vi "Create Groups.vi"(7 "Group":bool, 8 "error in (no error)":errorcluster, 11 "Channels":T1[](array[typedef]) {"Data Type" format="%.0x"}) -> (0 "error out":errorcluster, 3 "Channels out":T1[](array[typedef]) {"Data Type" format="%.0x"})   [LabVIEW 2020, in "FPGA Addon System Explorer.lvlib"]
uses:
  FPGA Addon System Explorer.lvlib
  Addon Shared/Types/Register Information.ctl
  Addon Shared/Types/FPGA Addon Data Type.ctl
  Addon Shared/FPGA Addon Shared.lvlib
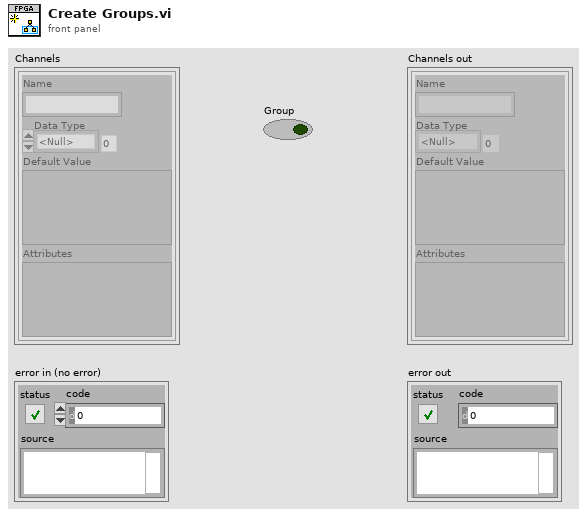
[diagram p1: front panel]
types:
  T1 = typedef "FPGA Addon Shared.lvlib/Register Information.ctl" = cluster{"Name":string, "Data Type":T2, "Default Value":variant, "Attributes":variant}
  T2 = typedef "FPGA Addon Shared.lvlib/FPGA Addon Data Type.ctl" = enum8{"<Null>", "I8", "I16", "I32", "I64", "U8", "U16", "U32", "U64", "SGL", "Boolean", "Analog PWM In Settings", "Analog PWM In", "Digital PWM In Settings", "Digital PWM In", "Digital PWM Out", "Sine Out", "FXP", "FXP+/-24.5", "FXP+/-16.5", "FXP+/-32.8", "FXP+/-64.32", "FXP+/-16.7", "FXP+/-20.5", "FXP+/-27.5", "FXP+/-32.16", "FXP+16.3", "FXP+18.3", "Digital Static In", "Digital Static Out", "Digital Static In Settings", "Digital WSS Out", "Quad Encoder Settings", "Quad Encoder In", "Group"}
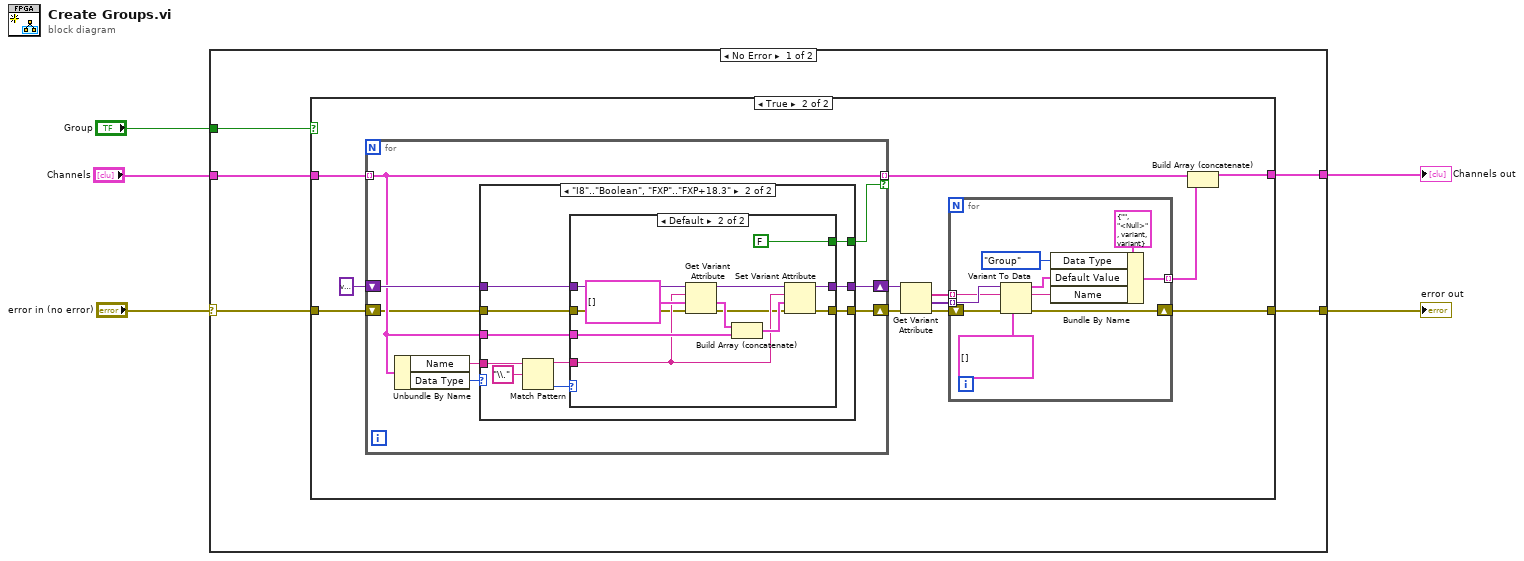
[diagram p0: block diagram]
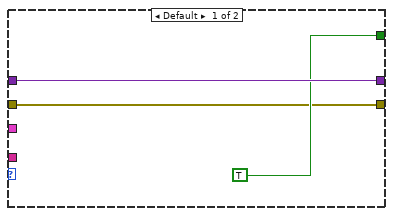
[diagram p3: hidden frame]
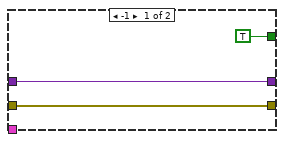
[diagram p4: hidden frame]
diagram:
  n1 = case shown="No Error" "error in (no error)" {
    selector: "error in (no error)" -> [w6 w70]
    tunnel: [w10 w71] -> w5
    tunnel: "Channels" -> [w9 w71]
    tunnel: [w8 w70] -> w3
    tunnel: "Group" -> [w7 _]
    frame No Error {
      n2 = case shown="True" w7 {
        tunnel: w9 -> [w11 w24]
        tunnel: w6 -> [w12 w17]
        tunnel: [w12 w16] -> w8
        tunnel: [w11 w15] -> w10
        frame False {
        }
        frame True {
          n3 = for {
            tunnel: w24 -> [w37] mode=indexing
            shift-right: [w38] -> w22
            shift-left: variant -> [w39]
            tunnel: [w37] -> w14 mode=indexing if=w36
            shift-right: [w35] -> w19
            shift-left: w17 -> [w34]
            n4 = Unbundle By Name(w37) -> ("Name"=w41:string, "Data Type"=w40:T2)
            n5 = case shown="\"I8\"..\"Boolean\", \"FXP\"..\"FXP+18.3\"" w40 {
              tunnel: w41 -> [_ w54]
              tunnel: w39 -> [w44 w51]
              tunnel: w37 -> [_ w49]
              tunnel: [w44 w48] -> w38
              tunnel: [TRUE w47] -> w36
              tunnel: [w42 w46] -> w35
              tunnel: w34 -> [w42 w45]
              frame Default {
              }
              frame "I8".."Boolean", "FXP".."FXP+18.3" {
                n6 = Match Pattern(string=w54, regular expression="\\.") -> (before substring=w50:string, offset past match=w52:i32)  [unwired: 1 in, 2 out]
                n7 = case shown="Default" w52 {
                  tunnel: w51 -> [w57 w69]
                  tunnel: w50 -> [_ w64]
                  tunnel: w49 -> [_ w66]
                  tunnel: [w57 w63] -> w48
                  tunnel: [TRUE FALSE] -> w47
                  tunnel: [w55 w61] -> w46
                  tunnel: w45 -> [w55 w60]
                  frame -1 {
                  }
                  frame Default {
                    n8 = Get Variant Attribute(Variant=w69, name=w64, default value (empty Variant)=T1[] [], error in=w60) -> (duplicate Variant=w58:variant, value=w67:T1[], error out=w59:errorcluster)  [unwired: 1 out]
                    n9 = Build Array (concatenate)(w67, w66) -> (w65:T1[])
                    n10 = Set Variant Attribute(Variant=w58, name=w64, value=w65, error in=w59) -> (Variant out=w63:variant, error out=w61:errorcluster)  [unwired: 1 out]
                  }
                }
              }
            }
          }
          n11 = Get Variant Attribute(Variant=w22, error in=w19) -> (names=w21:string[], values=w20:variant[], error out=w18:errorcluster)  [unwired: 2 in, 1 out]
          n12 = for {
            tunnel: w21 -> [w25] mode=indexing
            tunnel: w20 -> [w33] mode=indexing
            tunnel: [w28] -> w13 mode=indexing
            shift-right: [w26] -> w16
            shift-left: w18 -> [w27]
            n13 = Variant To Data(error in=w27, type=T1[] [], Variant=w33) -> (data=w29:T1[], error out=w26:errorcluster)
            n14 = Bundle By Name(cluster=T1 {"Name"="", "Data Type"=enum."<Null>", "Default Value"=variant, "Attributes"=variant}, "Data Type"=FPGA_Addon_Data_Type."Group", "Default Value"=w29, "Name"=w25) -> (w28:T1)
          }
          n15 = Build Array (concatenate)(w14, w13) -> (w15:T1[])
        }
      }
    }
    frame Error {
    }
  }
  "Channels out" <- w5
  "error out" <- w3
